vi "Parse Parameters File.vi"(8 "error in":errorcluster, 11 "path to XML document":path caption="path to parameters xml") -> (0 "error out":errorcluster, 1 "ports":T1[](array[typedef]), 3 "path to XML document out":path caption="path to parameters xml")   [LabVIEW 2021, in "ARINC 429 Import.lvlib"]
uses:
  ARINC 429 Import.lvlib
  Shared/VS Channels Definition for All Labels on Hardware Channel.ctl
  Shared/Direction.ctl
  Shared/VS Channels Definition for Label.ctl
  Shared/VS Channel Definition for Parameter.ctl
  Shared/Parameter Definition.ctl
  <vilib>/NI/NI VeriStand Encoding and Decoding/Encoding.ctl
  Shared/Transfer Type.ctl
  Shared/Transfer Speed.ctl
  c4e6e99b-49b2-4722-a2ba-8003c4091ae8.vi
  <vilib>/xml/Load XML File.vi
  Read Tag Element (U16).vi
  Read Tag Element (Speed).vi
  Read Tag Element (Direction).vi
  <vilib>/xml/Close Reference(Node).vi
  <vilib>/Comparison/Less/Less Functor/Less Functor.lvclass
  <vilib>/xml/NI_XML.lvlib
  <resource>/objmgr/DOMUserDefRef.rc
  <vilib>/NI/NI VeriStand Encoding and Decoding/Encoding and Decoding.lvlib
panel:
  out "parse errors":string
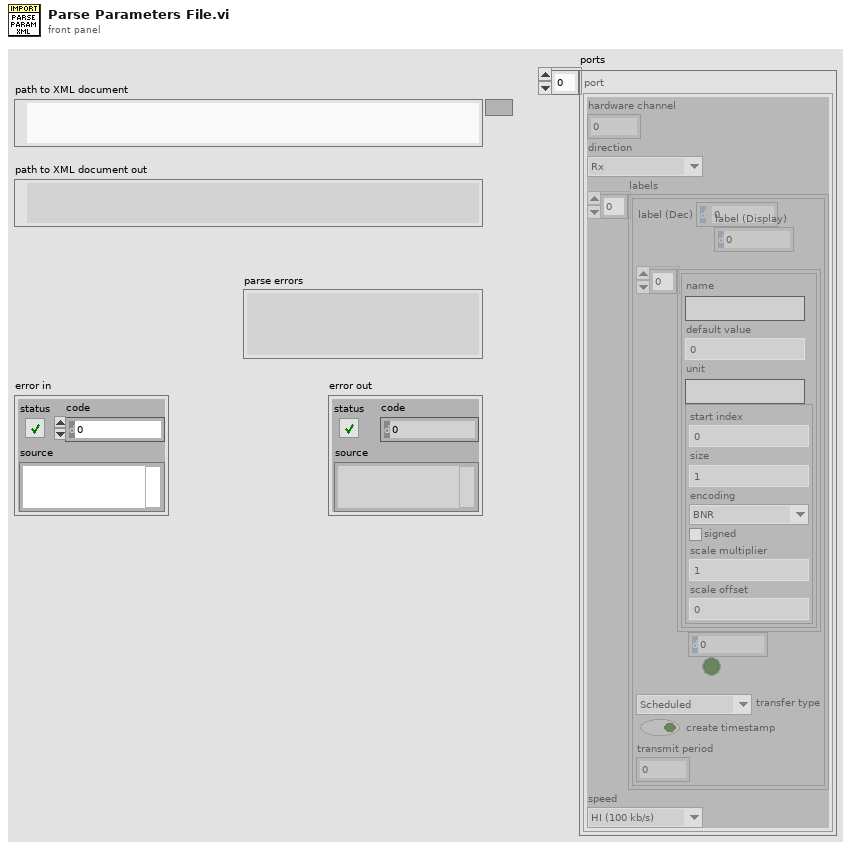
[diagram p1: front panel]
types:
  T1 = typedef "VS Channels Definition for All Labels on Hardware Channel.ctl" = cluster{"hardware channel":i32, "direction":T2, "labels":T3[], "speed":T8}
  T2 = typedef "Direction.ctl" = enum16{"Rx", "Tx"}
  T3 = typedef "VS Channels Definition for Label.ctl" = cluster{"label (Dec)":u32, "label (Display)":u32, "parameters":T4[], "SDI value":u8, "SDI enabled":bool, "transfer type":T7, "create timestamp":bool, "transmit period":u32}
  T4 = typedef "VS Channel Definition for Parameter.ctl" = cluster{"name":string, "default value":dbl, "unit":string, "Parameter":T5}
  T5 = typedef "Parameter Definition.ctl" = cluster{"start index":i32, "size":i32, "encoding":T6, "signed":bool, "scale multiplier":dbl, "scale offset":dbl}
  T6 = typedef "Encoding and Decoding.lvlib/Encoding.ctl" = enum16{"BNR", "BCD", "Discrete"}
  T7 = typedef "Transfer Type.ctl" = enum16{"Scheduled", "Acyclic", "Block", "Strobe"}
  T8 = typedef "Transfer Speed.ctl" = enum16{"LO (12.5 kb/s)", "HI (100 kb/s)"}
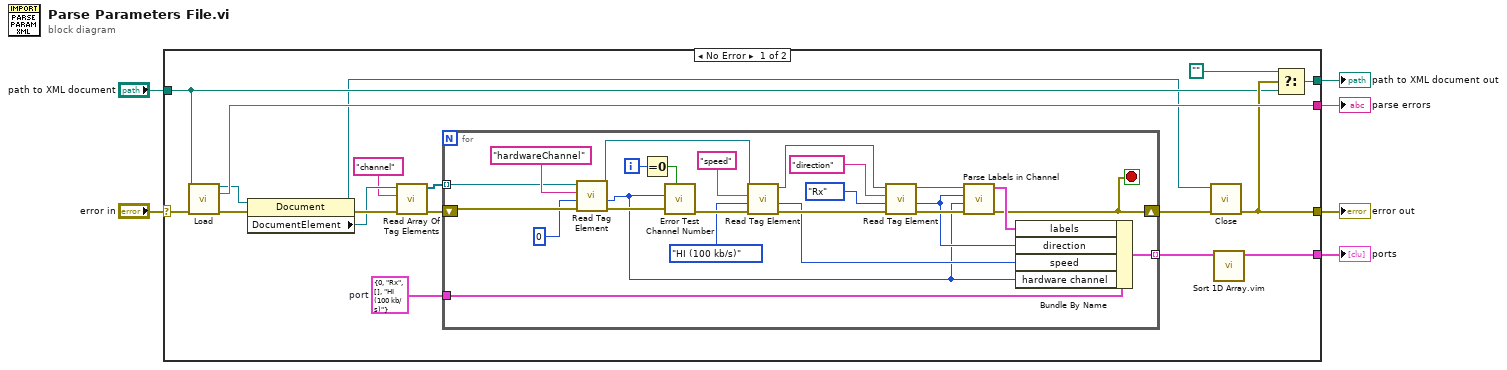
[diagram p0: block diagram]
diagram:
  n1 = case shown="No Error" "error in" {
    selector: "error in" -> [w23 w49]
    tunnel: [w24 _] -> w6
    tunnel: [w22 w49] -> w5
    tunnel: "path to XML document" -> [w20 _]
    tunnel: [w21 _] -> w2
    tunnel: [w11 _] -> w1
    frame No Error {
      w8 = T1 {"hardware channel"=0, "direction"=enum."Rx", "labels"=[], "speed"=enum."HI (100 kb/s)"}  # port
      n2 = call-poly <vilib>:"Load.vi"("path to XML document"=w20, "error in (no error)"=w23) -> ("DOM document out"=w18:refnum<k20>, "parse errors"=w24:string, "error out"=w17:errorcluster)  [unwired: 11 in]
      n3 = property class="Document"(reference=w18, error in=w17) -> (reference out=w10:refnum<k20>, error out=w16:errorcluster, "DocumentElement"=w15:refnum<k20>)
      n4 = call "Read Array Of Tag Elements.vi"("error in"=w16, "tag name"="channel" ("Tag Name"), "node in"=w15) -> ("error out"=w12:errorcluster, "array of elements"=w13:refnum<k20>[])  [unwired: 7 in]
      n5 = for {
        shift-right: [w25] -> w9
        shift-left: w12 -> [w33]
        tunnel: w8 -> [w40]
        tunnel: w13 -> [w29] mode=indexing
        tunnel: [w26] -> w7 mode=indexing
        i -> [w43]
        stop <- w25 stop-if-true
        n6 = call-poly "Read Tag Element.vi"("error in"=w33, "default"=u16 0, "Tag Name"="hardwareChannel", "node in"=w29) -> ("error out"=w32:errorcluster, "value"=w31:u16, "node out"=w27:refnum<k20>)  [unwired: 5 in]
        n7 = Equal To 0?(x=w43) -> (x = 0?=w42:bool)
        n8 = call "Error Test Channel Number.vi"("reset (F)"=w42, "error in"=w32, "channel #"=w31) -> ("error out"=w39:errorcluster)  [unwired: 8 in]
        n9 = call-poly "Read Tag Element.vi"("error in"=w39, "default"=Transfer_Speed."HI (100 kb/s)", "Tag Name"="speed", "node in"=w27) -> ("error out"=w38:errorcluster, "value"=w34:T8, "node out"=w35:refnum<k20>)  [unwired: 5 in]
        n10 = call-poly "Read Tag Element.vi"("error in"=w38, "default"=Direction."Rx", "Tag Name"="direction", "node in"=w35) -> ("error out"=w47:errorcluster, "value"=w41:T2, "node out"=w46:refnum<k20>)  [unwired: 5 in]
        n11 = call "Parse Labels in Channel.vi"("error in"=w47, "channel #"=w31, "direction"=w41, "node in"=w46) -> ("error out"=w25:errorcluster, "labels"=w45:T3[])  [unwired: 6 in]
        n12 = Bundle By Name(cluster=w40, "labels"=w45, "direction"=w41, "speed"=w34, "hardware channel"=w31) -> (w26:T1)
      }
      n13 = call-poly <vilib>:"Close.vi"("error in (no error)"=w9, "node"=w10) -> ("error out"=w22:errorcluster)  [unwired: 7 in]
      n14 = call "Sort 1D Array.vim"("unsorted array"=w7) -> ("sorted array"=w11:T1[])  [unwired: 10 in]
      n15 = Select(t=path "", s=w22, f=w20) -> (s? t:f=w21:path)
    }
    frame Error {
    }
  }
  "parse errors" <- w6
  "ports" <- w1
  "error out" <- w5
  "path to XML document out" <- w2
